vi "FuncVI_Sub - VI - preparation to run VI.vi"(8 "error in":errorcluster, 11 "VI name or path":string) -> (0 "error out":errorcluster, 1 "Exec.State":T1(ring), 3 "VI Refnum":refnum<vi>)   [LabVIEW 2021]
doc: "::: CalcExpress Toolkit :::\nCopyright (c) 2000-2026 Konstantin Shifershteyn. All rights reserved."
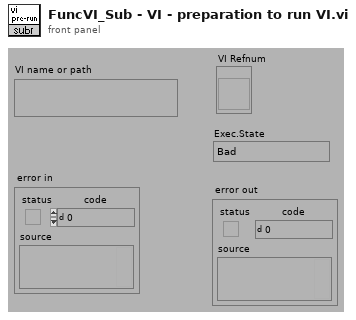
[diagram p1: front panel]
types:
  T1 = enum32{"Bad", "Idle", "Run top level", "Running"}
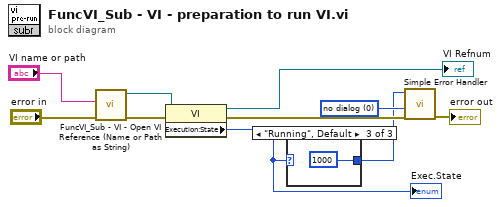
[diagram p0: block diagram]
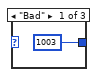
[diagram p2: hidden frame]
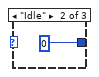
[diagram p3: hidden frame]
diagram:
  w8 = 0 items=["no dialog", "OK message", "continue or stop message"] ("type of dialog (OK msg:1)")
  n1 = call "FuncVI_Sub - VI - Open VI Reference (Name or Path as String).vi"("error in"="error in", "VI name or path"="VI name or path") -> ("error out"=w3:errorcluster, "VI Refnum"=w4:refnum<vi>)  [unwired: 8 in]
  n2 = property class="VI"(reference=w4, error in=w3) -> (reference out=→"VI Refnum":refnum<vi>, error out=w9:errorcluster, "Execution:State"=w6:T1)
  "Exec.State" <- w6
  n3 = case shown="\"Running\", Default" w6 {
    tunnel: [1003 0 1000] -> w7
    frame "Bad" {
    }
    frame "Idle" {
    }
    frame "Running", Default {
    }
  }
  n4 = call <vilib>:"Simple Error Handler.vi"("error code (no error:0)"=w7, "type of dialog (OK msg:1)"=w8, "error in (no error)"=w9) -> ("error out"=→"error out":errorcluster)  [unwired: 2 in, 4 out]
